vi "MenuHandler.vi"(5 "tree control":refnum<vi>, 7 "main message queue":T1, 8 "error in":errorcluster, 9 "parameters":variant, 10 "menu string":string, 11 "NISE_CEF_serializable node in":refnum<class "NISE_CEF_serializable node.lvclass">) -> (0 "error out":errorcluster, 1 "refresh tree?":bool, 2 "Unhandled":bool, 3 "NISE_CEF_serializable node out":refnum<class "NISE_CEF_serializable node.lvclass">)   [LabVIEW 2014, in "NISE_CEF_serializable node.lvclass"]
uses:
  NISE_CEF_serializable node.lvclass
  <vilib>/NI/AMC/Message Queue.ctl
  <vilib>/NI/AMC/Message.ctl
  <vilib>/NI/Tools/Keyed Array/KeyedArray.ctl
  Node/NISE_CEF_Node.lvclass
  <vilib>/NI/Tools/Keyed Array/Tools_KeyedArray.lvlib
  <vilib>/NI/AMC/AMC.lvlib
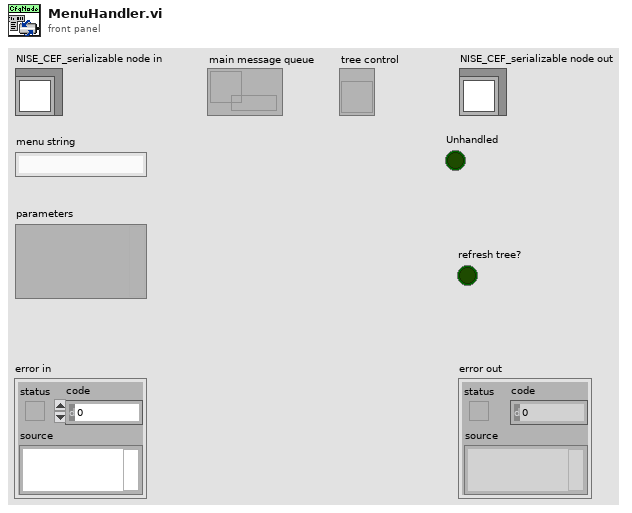
[diagram p1: front panel]
types:
  T1 = typedef "AMC.lvlib/Message Queue.ctl" = refnum<queue>
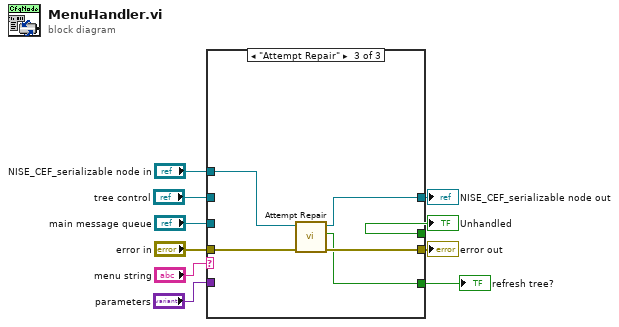
[diagram p0: block diagram]
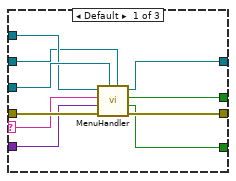
[diagram p2: hidden frame]
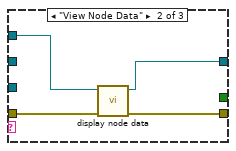
[diagram p3: hidden frame]
diagram:
  n1 = case shown="\"Attempt Repair\"" "menu string" {
    selector: "menu string" -> [w12 _ _]
    tunnel: [w18 _ _] -> w6
    tunnel: "NISE_CEF_serializable node in" -> [w16 w24 w26]
    tunnel: [w15 w23 w27] -> w9
    tunnel: [w19 w22 w28] -> w5
    tunnel: "error in" -> [w20 w21 w29]
    tunnel: "main message queue" -> [w17 _ _]
    tunnel: "parameters" -> [w14 _ _]
    tunnel: "tree control" -> [w13 _ _]
    tunnel: [w11 _ w25] -> w1
    frame Default {
      n2 = call-parent "MenuHandler.vi"("tree control"=w13, "main message queue"=w17, "error in"=w20, "parameters"=w14, "menu string"=w12, "NISE_CEF_Node in"=w16) -> ("error out"=w19:errorcluster, "refresh tree?"=w11:bool, "Unhandled"=w18:bool, "NISE_CEF_Node out"=w15:refnum<class "NISE_CEF_serializable node.lvclass">)  [unwired: 2 in]
    }
    frame "View Node Data" {
      n3 = call-dynamic "display node data.vi"("error in"=w21, "NISE_CEF_serializable node in"=w24) -> ("error out"=w22:errorcluster, "NISE_CEF_serializable node out"=w23:refnum<class "NISE_CEF_serializable node.lvclass">)  [unwired: 8 in]
    }
    frame "Attempt Repair" {
      n4 = call "Attempt Repair.vi"("error in"=w29, "NISE_CEF_serializable node in"=w26) -> ("error out"=w28:errorcluster, "refresh tree?"=w25:bool, "NISE_CEF_serializable node out"=w27:refnum<class "NISE_CEF_serializable node.lvclass">)  [unwired: 7 in]
    }
  }
  "error out" <- w5
  "NISE_CEF_serializable node out" <- w9
  "Unhandled" <- w6
  "refresh tree?" <- w1
